vi "Add OutputOffset to Offset.vi"(8 "error in (no error)":errorcluster, 11 "Instrument.DAQ":refnum<class "Instrument.DAQ.lvclass">) -> (0 "error out":errorcluster, 3 "Instrument.DAQ out":refnum<class "Instrument.DAQ.lvclass">)   [LabVIEW 2019, in "Instrument.Lockin.lvlib" / "Instrument.DAQ.lvclass"]
uses:
  Instrument.DAQ.lvclass
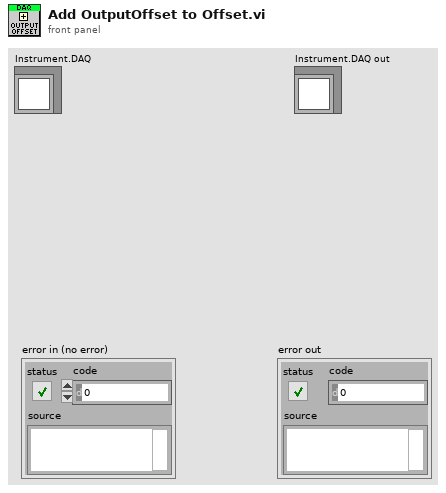
[diagram p1: front panel]
types:
  T1 = typedef "Instrument.Lockin.lvlib/Instrument.DAQ.lvclass/AO.Channel--Cluster--Array.ctl" = T2[]
  T2 = typedef "Instrument.Lockin.lvlib/Instrument.DAQ.lvclass/AO.Channel--Cluster.ctl" = cluster{"Enable?":bool, "Channel":i32, "Amplitude":dbl, "Offset":dbl, "Frequency":dbl, "Phase":dbl, "Function":T3, "Sweeping?":bool, "Limit AC":bool, "Limit DC?":bool, "Duty Cycle":bool}
  T3 = typedef "Instrument.Lockin.lvlib/Instrument.DAQ.lvclass/AO.Channel.Function--Enum.ctl" = enum16{"sine", "square", "triangle", "saw"}
  T4 = typedef "Instrument.Lockin.lvlib/Instrument.DAQ.lvclass/Channel.Offset--Cluster--Array.ctl" = T5[]
  T5 = typedef "Instrument.Lockin.lvlib/Instrument.DAQ.lvclass/Channel.Offset--Cluster.ctl" = cluster{"Channel":string, "Offset":dbl}
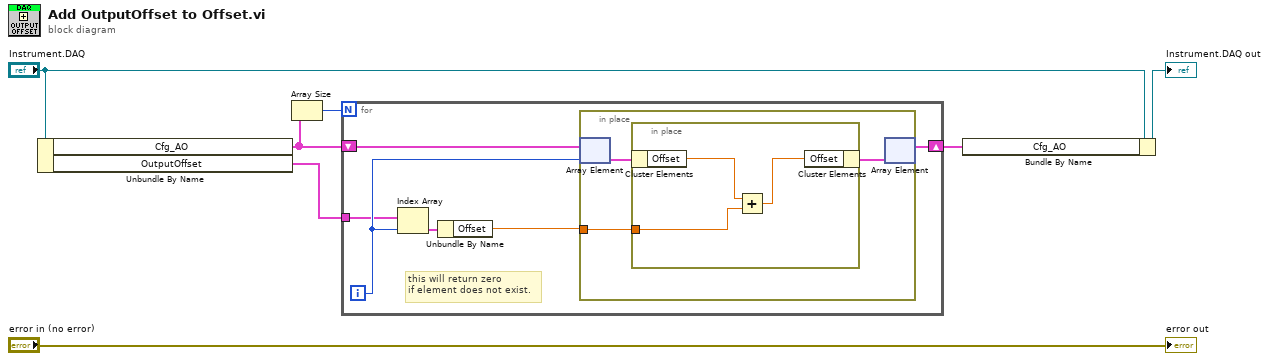
[diagram p0: block diagram]
diagram:
  n1 = Unbundle By Name("Instrument.DAQ") -> ("Cfg_AO"=w5:T1, "OutputOffset"=w1:T4)
  n2 = Array Size(array=w5) -> (size(s)=w6:i32)
  n3 = for {
    N: w6 -> [_]
    tunnel: w1 -> [w10]
    shift-right: [w13] -> w2
    shift-left: w5 -> [w11]
    i -> [w12]
    # "this will return zero\nif element does not exist."
    n4 = Index Array(array=w10, index=w12) -> (element=w9:T5)
    n5 = Unbundle By Name(w9) -> ("Offset"=w8:dbl)
    n6 = in-place {
      in-place-border: w8 -> [w16]
      n7 = in-place-array #1(w11, w12) -> (w14:T2)
      n8 = in-place {
        in-place-border: w16 -> [w18]
        n9 = in-place-cluster #2(w14) -> ("Offset"=w19:dbl)
        n10 = Add(x=w19, y=w18) -> (x+y=w17:dbl)
        n11 = in-place-cluster #2("Offset"=w17) -> (w15:T2)
      }
      n12 = in-place-array #1(w15) -> (w13:T1)  [unwired: 1 out]
    }
  }
  n13 = Bundle By Name(cluster="Instrument.DAQ", "Cfg_AO"=w2) -> (→"Instrument.DAQ out":refnum<class "Instrument.DAQ.lvclass">)
  "error out" <- "error in (no error)"
